vi "Check If Environment Variable Exists.vi"(7 "Target (Process)":T1 items=["Process", "User", "Machine"], 8 "Error In":errorcluster, 11 "Name":string) -> (0 "Error Out":errorcluster, 3 "Exists?":bool)   [LabVIEW 2019, in "SLL Environment Variable.lvlib"]
doc: "Check if the environment variable exists in <B>Target</B> environment."
uses:
  SLL Environment Variable.lvlib
  _Typedef/Target Environment Enum.ctl
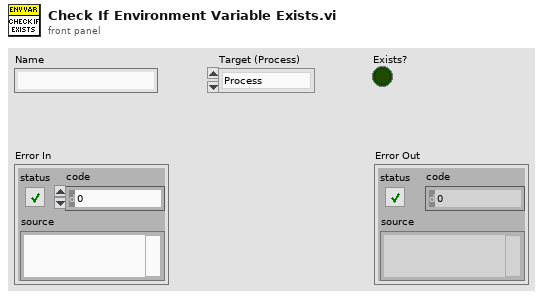
[diagram p1: front panel]
types:
  T1 = typedef "SLL Environment Variable.lvlib/Target Environment Enum.ctl" = i32
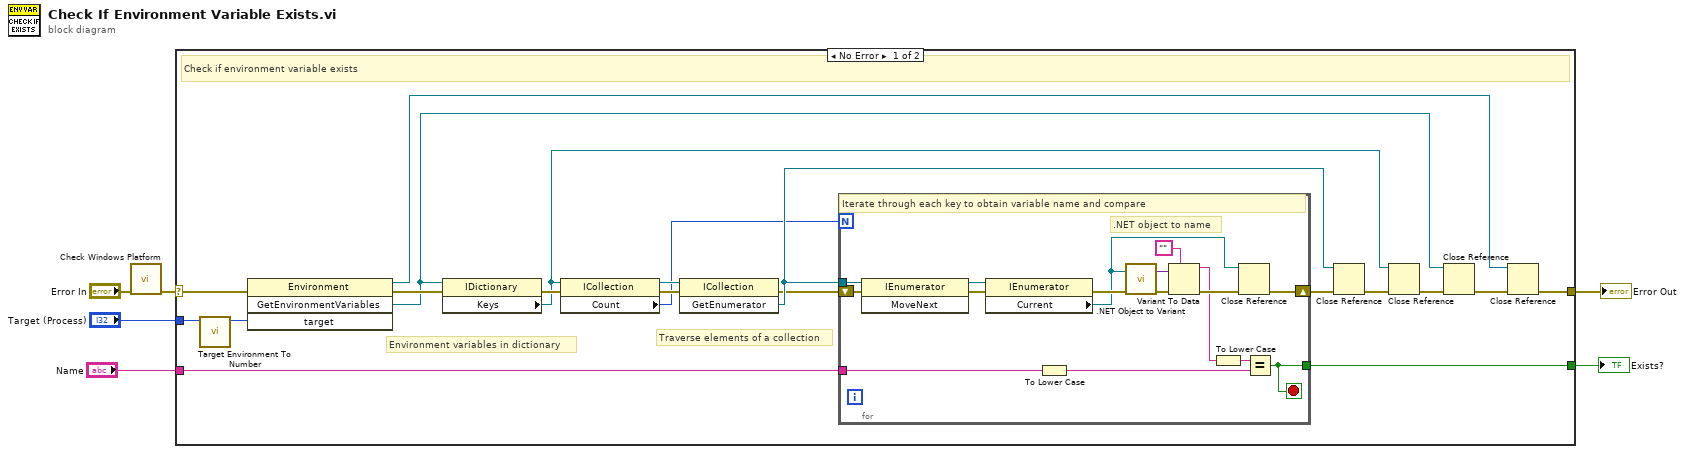
[diagram p0: block diagram]
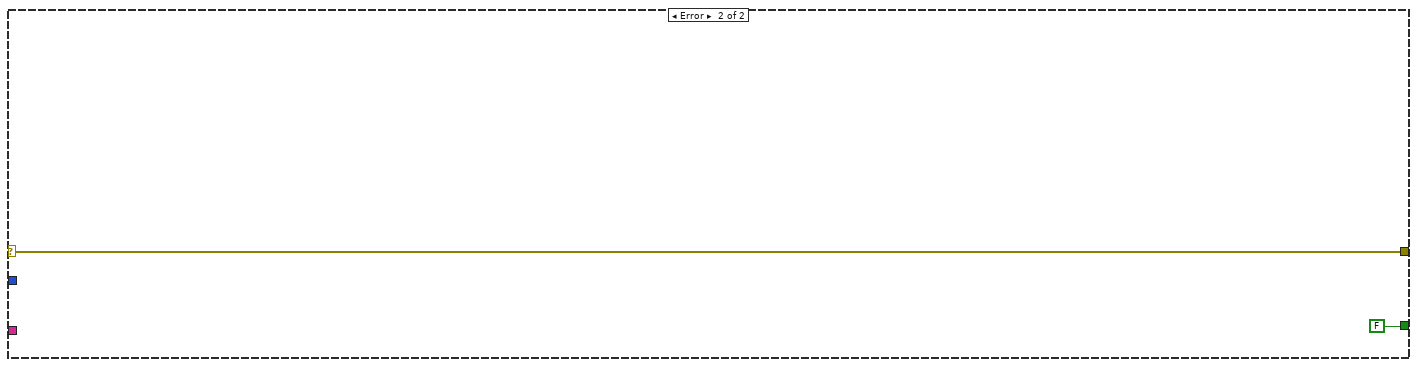
[diagram p2: hidden frame]
diagram:
  n1 = call "Check Windows Platform.vi"("Error In"="Error In") -> ("Error Out"=w6:errorcluster)  [unwired: 10 in]
  n2 = case shown="No Error" w6 {
    selector: w6 -> [w11 w44]
    tunnel: [w15 w44] -> w3
    tunnel: "Target (Process)" -> [w10 _]
    tunnel: "Name" -> [w8 _]
    tunnel: [w7 FALSE] -> w1
    frame No Error {
      # "Traverse elements of a collection"
      # "Environment variables in dictionary"
      # "Check if environment variable exists"
      n3 = call "Target Environment To Number.vi"("Target (Process)"=w10) -> ("Numeric Value"=w9:i32)  [unwired: 10 in]
      n4 = invoke class="Environment" method="GetEnvironmentVariables"(error in=w11, "target"=w9) -> (reference out=w14:refnum<k24>, error out=w17:errorcluster, "GetEnvironmentVariables"=w16:refnum<k24>)  [unwired: 2 in, 1 out]
      n5 = property class="IDictionary"(reference=w16, error in=w17) -> (error out=w18:errorcluster, "Keys"=w13:refnum<k24>)  [unwired: 1 out]
      n6 = property class="ICollection"(reference=w13, error in=w18) -> (reference out=w20:refnum<k24>, error out=w19:errorcluster, "Count"=w12:i32)
      n7 = invoke class="ICollection" method="GetEnumerator"(reference=w20, error in=w19) -> (error out=w21:errorcluster, "GetEnumerator"=w22:refnum<k24>)  [unwired: 1 in, 1 out]
      n8 = for {
        N: w12 -> [_]
        tunnel: w22 -> [w39]
        shift-right: [w41] -> w26
        shift-left: w21 -> [w42]
        tunnel: w8 -> [w30]
        tunnel: [w27] -> w7
        stop <- w27 stop-if-true
        # ".NET object to name"
        # "Iterate through each key to obtain variable name and compare"
        n9 = invoke class="IEnumerator" method="MoveNext"(reference=w39, error in=w42) -> (reference out=w32:refnum<k24>, error out=w40:errorcluster)  [unwired: 1 in, 1 out]
        n10 = property class="IEnumerator"(reference=w32, error in=w40) -> (error out=w38:errorcluster, "Current"=w33:refnum<k24>)  [unwired: 1 out]
        n11 = To Lower Case(string=w30) -> (all lower case string=w29:string)
        n12 = call <vilib>:".NET Object to Variant.vi"("error in (no error)"=w38, ".NET object"=w33) -> ("error out"=w37:errorcluster, "variant"=w36:variant)
        n13 = Variant To Data(error in=w37, type="", Variant=w36) -> (data=w31:string, error out=w35:errorcluster)
        n14 = To Lower Case(string=w31) -> (all lower case string=w28:string)
        n15 = Close Reference(reference=w33, error in (no error)=w35) -> (error out=w41:errorcluster)
        n16 = Equal?(x=w28, y=w29) -> (x = y?=w27:bool)
      }
      n17 = Close Reference(reference=w22, error in (no error)=w26) -> (error out=w23:errorcluster)
      n18 = Close Reference(reference=w13, error in (no error)=w23) -> (error out=w24:errorcluster)
      n19 = Close Reference(reference=w16, error in (no error)=w24) -> (error out=w25:errorcluster)
      n20 = Close Reference(reference=w14, error in (no error)=w25) -> (error out=w15:errorcluster)
    }
    frame Error {
    }
  }
  "Error Out" <- w3
  "Exists?" <- w1
